vi "Parameters_Build_Reference.vi"(10 "Reference Move Parameters":T1={"Reference Move Mode"=11599899, "Start Search Forward"=FALSE, "Stop on FWD Edge"=FALSE, "Approach Forward"=FALSE, "Velocity"=0.0, "Acceleration"=0.0} {"Reference Move Mode" items=["Home"=11599899, "Index"=11599900, "Center"=11599901, "Forward Limit"=11599902, "Reverse Limit"=11599903, "Absolute"=12648450]}, 11 "Axis to command":i32) -> (3 "Parameters":dbl[](array[numeric]))   [LabVIEW 2017, in "WordManipulationLibrary.lvlib"]
uses:
  WordManipulationLibrary.lvlib
  Parameters_Reference.ctl
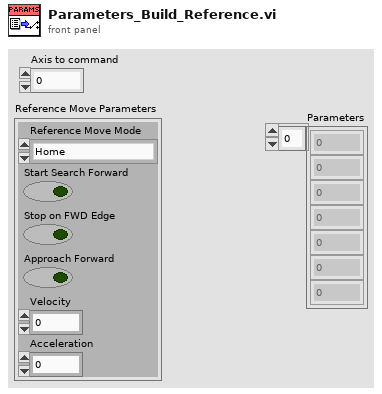
[diagram p1: front panel]
types:
  T1 = typedef "WordManipulationLibrary.lvlib/Parameters_Reference.ctl" = cluster{"Reference Move Mode":i32, "Start Search Forward":bool, "Stop on FWD Edge":bool, "Approach Forward":bool, "Velocity":dbl, "Acceleration":dbl}
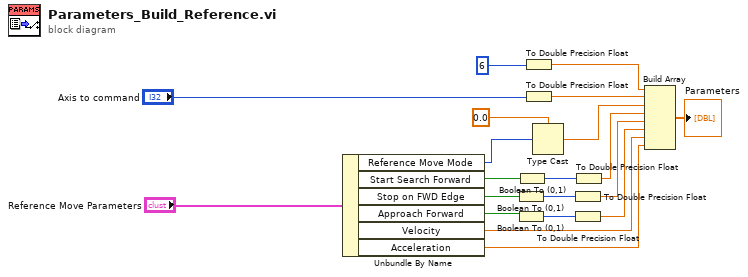
[diagram p0: block diagram]
diagram:
  n1 = Unbundle By Name("Reference Move Parameters") -> ("Reference Move Mode"=w3:i32, "Start Search Forward"=w19:bool, "Stop on FWD Edge"=w15:bool, "Approach Forward"=w14:bool, "Velocity"=w9:dbl, "Acceleration"=w8:dbl)
  n2 = Boolean To (0,1)(Boolean=w15) -> (0, 1=w17:i16)
  n3 = Boolean To (0,1)(Boolean=w14) -> (0, 1=w16:i16)
  n4 = Boolean To (0,1)(Boolean=w19) -> (0, 1=w18:i16)
  n5 = To Double Precision Float(number=i16 6 ("element")) -> (double precision float=w4:dbl)
  n6 = To Double Precision Float(number="Axis to command") -> (double precision float=w6:dbl)
  n7 = Type Cast(type=0.0 ("element"), x=w3) -> (*(type *) &x=w2:dbl)
  n8 = To Double Precision Float(number=w17) -> (double precision float=w11:dbl)
  n9 = To Double Precision Float(number=w16) -> (double precision float=w10:dbl)
  n10 = To Double Precision Float(number=w18) -> (double precision float=w12:dbl)
  n11 = Build Array(w4, w6, w2, w12, w11, w10, w9, w8) -> (→"Parameters":dbl[])
